vi "CE Client - Error Handler.vi"(6 "error before":errorcluster, 8 "error message":string, 9 "CE error status":bool) -> (0 "error out":errorcluster)   [LabVIEW 2021]
doc: "::: CalcExpress Toolkit :::\nCopyright (c) 2000-2026 Konstantin Shifershteyn. All rights reserved."
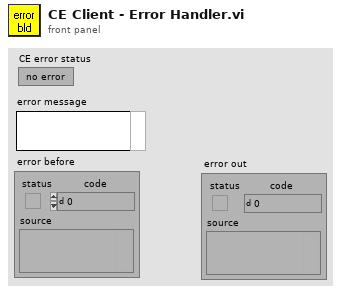
[diagram p1: front panel]
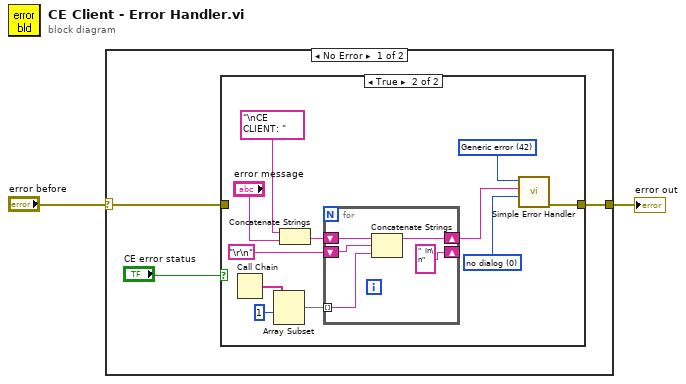
[diagram p0: block diagram]
diagram:
  n1 = case shown="No Error" "error before" {
    selector: "error before" -> [w3 w23]
    tunnel: [w5 w23] -> w2
    frame No Error {
      n2 = case shown="True" "CE error status" {
        tunnel: [w6 w11] -> w5
        tunnel: w3 -> [w6 _]
        frame False {
        }
        frame True {
          w7 = u16 42 items=["No error", "Argument error", "Memory is full", "Out of zone", "End of file", "File already open", "Generic file I/O error", "File not found", "File permission error", "Disk is full", "Duplicate path", "Too many files open", "System feature not enabled", "Resource file not found", "Cannot add resource", "Resource not found", "Image not found", "Image memory error", "Pen does not exist", "Config type invalid", "Config token not found", "Config parse error", "Config memory error", "Bad external code format", "Bad external code offset", "External code not present", "Null window", "Destroy window error", "Null menu", "Print aborted", "Bad print record", "Print driver error", "Windows error during printing", "Memory error during printing", "Print dialog error", "Generic print error", "Invalid device refnum", "Device not found", "Device parameter error", "Device unit error", "Cannot open device", "Device call aborted", "Generic error", "Cancelled by user", "Object ID too low", "Object ID too high", "Object not in heap", "Unknown heap", "Unknown object (invalid DefProc)", "Unknown object (DefProc not in table)", "Message out of range", "Invalid (null) method", "Unknown message", "Manager call not supported", "Bad address", "Network operation in progress", "Network operation timed out", "Connection is busy", "Network attribute not supported", "Network error", "Address in use", "System out of memory", "Connection aborted", "Connection refused", "Not connected", "Already connected", "Connection closed", "Initialization error (interapplication manager)", "Bad occurrence", "Wait on unbound occurrence handler", "Occurrence queue overflow", "Datalog type conflict", "Unused", "Unrecognized type (interapplication manager)", "Memory corrupt", "Failed to make temporary DLL", "Old CIN version", "Drag socket not found", "Failed to load drop-object", "Failed to register OLE object", "Failed to release OLE object", "Format specifier type mismatch", "Unknown format specifier", "Too few format specifiers", "Too many format specifiers", "Scan failed", "Newer CIN version", "OLE Convert", "Runtime menu error", "Password tampered", "Unknown error code"]
          w17 = 0 items=["no dialog", "OK message", "continue or stop message"] ("type of dialog (OK msg:1)")
          n3 = Call Chain() -> (call chain=w15:string[])
          n4 = Array Subset(array=w15, index=1) -> (w14:string[])  [unwired: 1 in]
          n5 = Concatenate Strings("\nCE CLIENT: " ("source"), "error message") -> (w8:string)
          n6 = for {
            shift-right: [w20] -> w12
            shift-left: w8 -> [w21]
            tunnel: w14 -> [w19] mode=indexing
            shift-right: ["  in\n"] -> _
            shift-left: "\r\n" -> [w18]
            n7 = Concatenate Strings(w21, w18, w19) -> (w20:string)
          }
          n8 = call <vilib>:"Simple Error Handler.vi"("error code (no error:0)"=w7, "error source (\" \")"=w12, "type of dialog (OK msg:1)"=w17) -> ("error out"=w11:errorcluster)  [unwired: 2 in, 4 out]
        }
      }
    }
    frame Error {
    }
  }
  "error out" <- w2
